vi "Sous_VI_Monter_Bras.vi"   [LabVIEW 2017]
uses:
  enum_bras.ctl
types:
  T1 = typedef "enum_bras.ctl" = enum16{"Depart Bras", "Clapet Bras", "Inactif Bras", "Seaux Bras"}
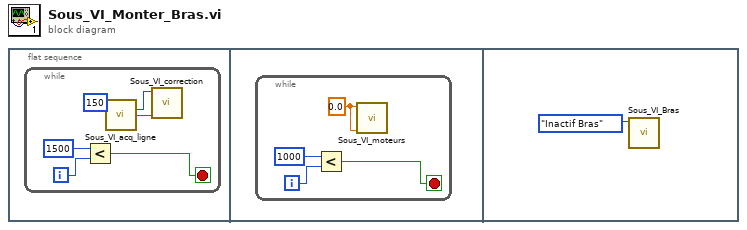
[diagram p0: block diagram]
diagram:
  n1 = flat-sequence {
    frame #0 {
      n2 = while {
        i -> [w6]
        stop <- w4 stop-if-true
        n3 = Less?(x=1500, y=w6) -> (x < y?=w4:bool)
        n4 = call "Sous_VI_acq_ligne.vi"("Seuil"=150) -> ("Décalage"=w3:u32, "G/D ?"=w2:bool)  [unwired: 10 in, 3 out]
        n5 = call "Sous_VI_correction.vi"("G/D ?"=w2, "Décalage"=w3) -> ()  [unwired: 10 in]
      }
    }
    frame #1 {
      n6 = while {
        i -> [w10]
        stop <- w8 stop-if-true
        w7 = 0.0 ("moteur gauche vite")
        n7 = Less?(x=1000, y=w10) -> (x < y?=w8:bool)
        n8 = call "Sous_VI_moteurs.vi"("Moteur Droit"=w7, "Moteur Gauche"=w7) -> ()  [unwired: 10 in]
      }
    }
    frame #2 {
      n9 = call "Sous_VI_Bras.vi"("Enum bras"=enum_bras."Inactif Bras") -> ()  [unwired: 11 in]
    }
  }
